vi "Write Elements.vi"(8 "error in":errorcluster, 10 "Elements":refnum<class "IElement.lvclass">[](array[class]), 11 "Type Definition in":refnum<class "Type Definition.lvclass">) -> (0 "error out":errorcluster, 3 "Type Definition out":refnum<class "Type Definition.lvclass">)   [LabVIEW 2026, in "Type Definition.lvclass"]
doc: "Data accessor."
uses:
  Type Definition.lvclass
  Interfaces/IElement/IElement.lvclass
  Type Definition.lvclass/Type Definition.ctl
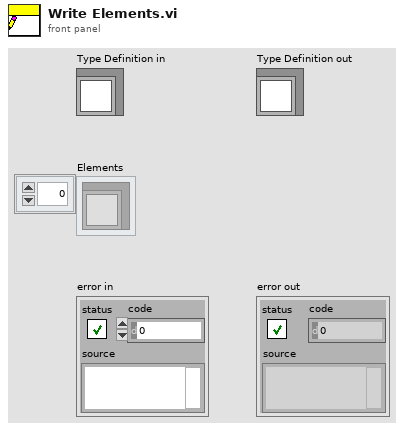
[diagram p1: front panel]
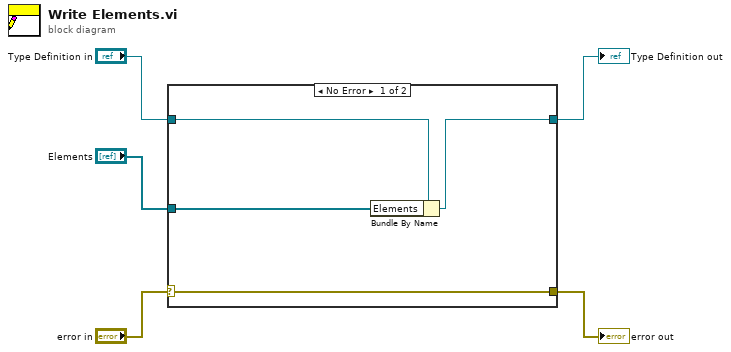
[diagram p0: block diagram]
diagram:
  n1 = case shown="No Error" "error in" {
    selector: "error in" -> [w9 w11]
    tunnel: [w9 w11] -> w4
    tunnel: [w7 w10] -> w2
    tunnel: "Type Definition in" -> [w8 w10]
    tunnel: "Elements" -> [w6 _]
    frame No Error {
      n2 = Bundle By Name(cluster=w8, "Elements"=w6) -> (w7:refnum<class "Type Definition.lvclass">)
    }
    frame Error {
      # "Pass error without further action."
    }
  }
  "error out" <- w4
  "Type Definition out" <- w2
